vi "Open Device.vi"(0 "transport_config":T1, 3 "error in":errorcluster) -> (5 "Session":T3, 8 "error out":errorcluster)   [LabVIEW 2015, in "Lengmur_socket.lvlib"]
uses:
  Lengmur_socket.lvlib
  Internal/Device Command.ctl
  Types/Device Config.ctl
  Types/Device Event.ctl
  Types/Measurement Point.ctl
  Types/Device Session.ctl
  Types/Transport Config.ctl
  Types/Transport Kind.ctl
panel:
  out "queue out 2":refnum<queue>
  out "queue out":refnum<queue>
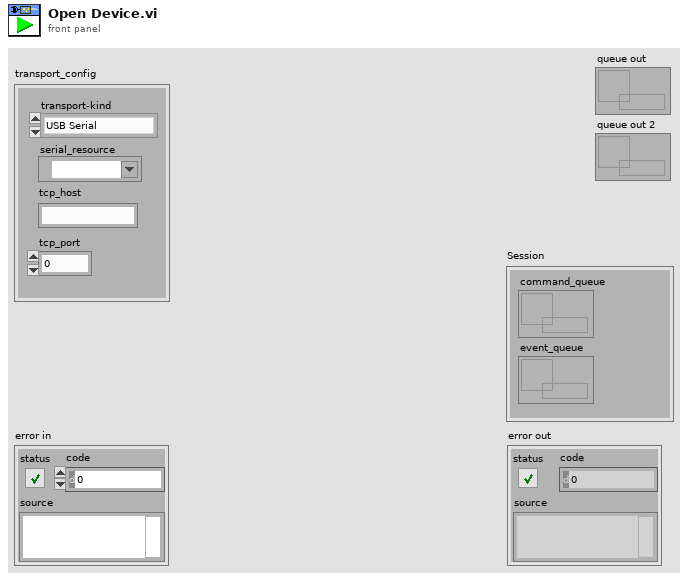
[diagram p1: front panel]
types:
  T1 = typedef "Lengmur_socket.lvlib/Transport Config.ctl" = cluster{"transport-kind":T2, "serial_resource":refnum<visa-resource-name>, "tcp_host":string, "tcp_port":u16}
  T2 = typedef "Lengmur_socket.lvlib/Transport Kind.ctl" = enum16{"USB Serial", "Ethernet TCP"}
  T3 = typedef "Lengmur_socket.lvlib/Device Session.ctl" = cluster{"command_queue":refnum<queue>, "event_queue":refnum<queue>}
  T4 = typedef "Lengmur_socket.lvlib/Device Event.ctl" = cluster{"event_type":enum16{"None", "Telemetry", "Command Response", "Sweep Complete", "Device Error", "Transport Error"}, "measurement":T5, "configuration":T6, "sweep_points":T5[], "command_ok":bool, "device_error":string, "error":errorcluster}
  T5 = typedef "Lengmur_socket.lvlib/Measurement Point.ctl" = cluster{"voltage_code":i16, "current_code":i16}
  T6 = typedef "Lengmur_socket.lvlib/Device Config.ctl" = cluster{"sample_rate":i32, "min_voltage":i32, "max_voltage":i32, "shunt_res":enum16{"auto", "200", "1000", "10000", "100000", "1000000", "10000000"}}
  T7 = typedef "Lengmur_socket.lvlib/Device Command.ctl" = cluster{"operation":enum16{"Get Configuration", "Set Configuration", "Start Sweep", "Shutdown"}, "configuration":T6}
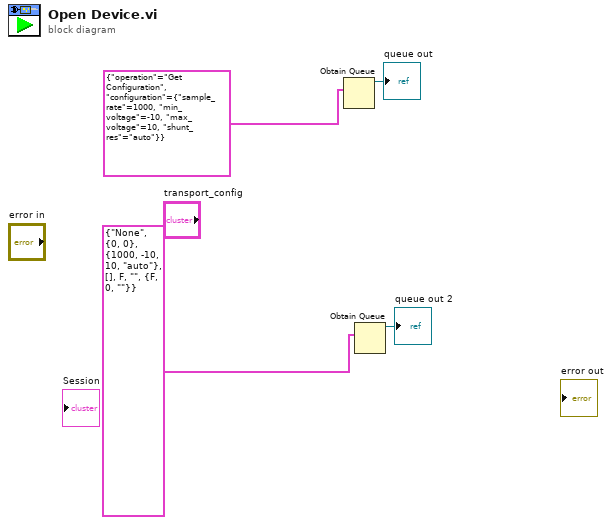
[diagram p0: block diagram]
diagram:
  n1 = Obtain Queue(element data type=T7 {"operation"=enum."Get Configuration", "configuration"={"sample_rate"=1000, "min_voltage"=-10, "max_voltage"=10, "shunt_res"=enum."auto"}} ("Device Command")) -> (queue out=→"queue out":refnum<queue>)  [unwired: 4 in, 2 out]
  n2 = Obtain Queue(element data type=T4 {"event_type"=enum."None", "measurement"={"voltage_code"=0, "current_code"=0}, "configuration"={"sample_rate"=1000, "min_voltage"=-10, "max_voltage"=10, "shunt_res"=enum."auto"}, "sweep_points"=[], "command_ok"=FALSE, "device_error"="", "error"={"status"=FALSE, "code"=0, "source"=""}} ("Device Event")) -> (queue out=→"queue out 2":refnum<queue>)  [unwired: 4 in, 2 out]
